vi "Read.vi"(8 "error in (no error)":errorcluster, 9 "timeout (ms)":i32=200, 10 "number to read":i32=100, 11 "XNET_CAN_RW in":refnum<class "XNET CAN RW.lvclass">) -> (0 "error out":errorcluster, 1 "Timeout":bool, 2 "pcap CAN Data":u8[](array[numeric]), 3 "XNET_CAN_RW out":refnum<class "XNET CAN RW.lvclass">, 4 "number read":i32=100)   [LabVIEW 2021, in "XNET CAN RW.lvclass"]
uses:
  XNET CAN RW.lvclass
  C:/Program Files/National Instruments/LabVIEW 2021/vi.lib/CIF Foundation/CIF CAN RW Core/CAN_RW_CORE.lvclass
  XNET CAN RW.lvclass/XNET CAN RW.ctl
  <vilib>/CIF Foundation/CIF CAN RW Core/CAN_RW_CORE.lvclass/CAN_RW_CORE.ctl
  Utilities/Get Time Pair.vi
  <vilib>/CIF Foundation/CIF CAN RW Core/Accessors/Read Statistcs.vi
  <vilib>/CIF Foundation/CIF CAN RW Core/Accessors/Write Statistcs.vi
  <vilib>/CIF Foundation/CIF Utilities/Time/System Time/LabVIEW Time to TAI Time.vi
  <vilib>/CIF Foundation/CIF Utilities/Time/System Time/Get System Time.vi
  <vilib>/xnet/xnet.llb/XNET Read (Frame CAN).vi
  <vilib>/xnet/xnet.llb/XNET Read (State Time Current).vi
  <vilib>/CIF Foundation/CIF CAN RW Core/CAN_RW_CORE.lvclass
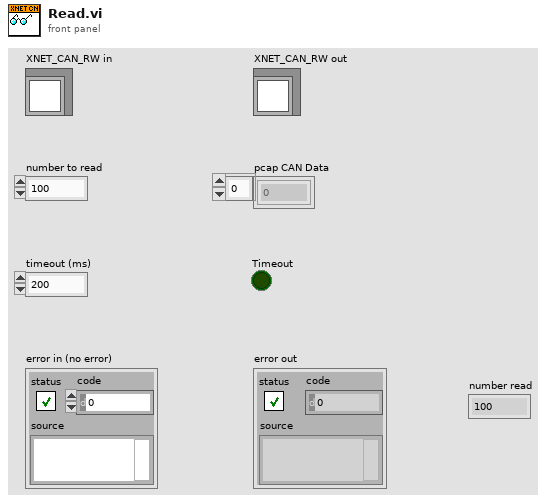
[diagram p1: front panel]
types:
  T1 = typedef "XNET Frame CAN.ctl" = cluster{"timestamp":timestamp, "payload":u8[], "identifier":u32, "type":T2, "extended?":bool, "echo?":bool}
  T2 = typedef "XNET Frame Type CAN.ctl" = u8
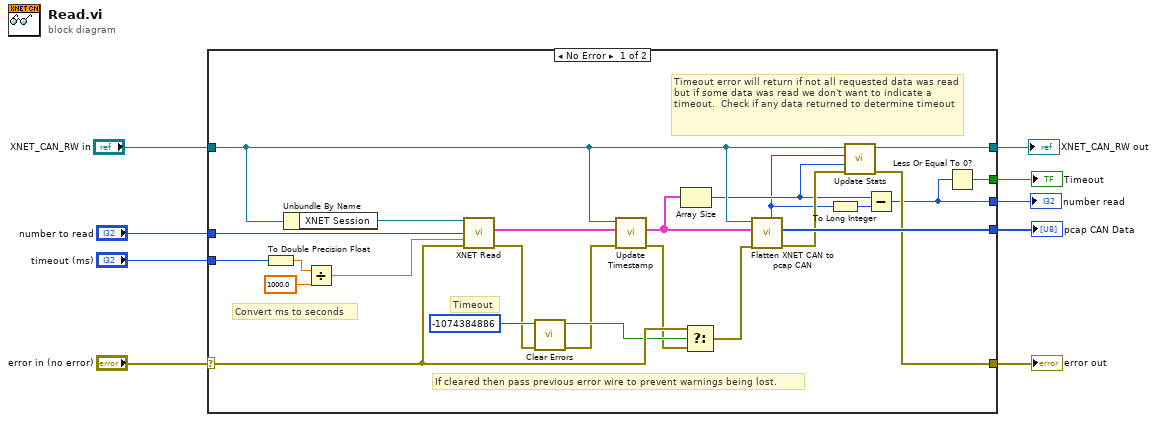
[diagram p0: block diagram]
diagram:
  n1 = case shown="No Error" "error in (no error)" {
    selector: "error in (no error)" -> [w27 w36]
    tunnel: [w19 w36] -> w8
    tunnel: [w20 w35] -> w6
    tunnel: "XNET_CAN_RW in" -> [w21 w35]
    tunnel: "timeout (ms)" -> [w30 _]
    tunnel: "number to read" -> [w29 _]
    tunnel: [w25 _] -> w3
    tunnel: [w22 _] -> w2
    tunnel: [w10 _] -> w1
    frame No Error {
      # "Timeout error will return if not all requested data was read but if some data was read we don't want to indicate a timeout.  Check if any data returned to determine timeout"
      # "Timeout"
      # "If cleared then pass previous error wire to prevent warnings being lost."
      # "Convert ms to seconds"
      n2 = To Double Precision Float(number=w30) -> (double precision float=w33:dbl)
      n3 = Unbundle By Name(w21) -> ("XNET Session"=w34:refnum<k21>)
      n4 = Divide(x=w33, y=1000.0) -> (x/y=w31:dbl)
      n5 = call-poly <vilib>:"XNET Read.vi"("session in"=w34, "number to read (-1)"=w29, "timeout (0)"=w31, "error in (no error)"=w27) -> ("data"=w24:T1[], "error out"=w16:errorcluster)  [unwired: 8 in, 2 out]
      n6 = call <vilib>:"Clear Errors.vi"("error in (no error)"=w16, "specific error code to clear (0: all)"=-1074384886) -> ("error out"=w15:errorcluster, "specific error cleared?"=w26:bool)  [unwired: 4 in]
      n7 = call "Update Timestamp.vi"("error in (no error)"=w15, "XNET CAN Data in"=w24, "XNET CAN RW in"=w21) -> ("error out"=w14:errorcluster, "XNET CAN Data out"=w23:T1[])  [unwired: 7 in]
      n8 = Array Size(array=w23) -> (size(s)=w13:i32)
      n9 = Select(t=w27, s=w26, f=w14) -> (s? t:f=w18:errorcluster)
      n10 = call "Flatten XNET CAN to pcap CAN.vi"("error in (no error)"=w18, "XNET CAN Data"=w23, "XNET_CAN_RW in"=w21) -> ("error out"=w17:errorcluster, "pcap CAN DATA"=w25:u8[], "Number Filtered"=w12:u32)  [unwired: 6 in]
      n11 = To Long Integer(number=w12) -> (32bit integer=w11:i32)
      n12 = call <vilib>:"Update Stats.vi"("error in (no error)"=w17, "Number Read"=w13, "Number Filtered"=w12, "CAN_RW_CORE in"=w21) -> ("error out"=w19:errorcluster, "CAN_RW_CORE out"=w20:refnum<class "XNET CAN RW.lvclass">)  [unwired: 6 in]
      n13 = Subtract(x=w13, y=w11) -> (x-y=w10:i32)
      n14 = Less Or Equal To 0?(x=w10) -> (x <= 0?=w22:bool)
    }
    frame Error {
    }
  }
  "error out" <- w8
  "XNET_CAN_RW out" <- w6
  "Timeout" <- w2
  "pcap CAN Data" <- w3
  "number read" <- w1
